vi "GateCrossing.vi"() -> ()   [LabVIEW 2024]
uses:
  class/mqtt/mqttTypedef/mqttSubscribeCluster.ctl
  class/mqtt/mqttTypedef/mqttQOSlevel.ctl
  class/mqtt/mqttTypedef/mqttBroker.ctl
  class/mqtt/mqttTypedef/mqttWillInformation.ctl
  class/mqtt/mqttTXqueue/mqttTXdataQueueFunction.ctl
  class/mqtt/mqttConfigFunction.ctl
  class/mqtt/mqttTXqueue/mqttRXsubscriptionEventFunction.ctl
  class/mqtt/mqttTypedef/mqttConnectionMeta.ctl
  <vilib>/Instr/_visa.llb/VISA Configure Serial Port (Instr).vi
  class/mqtt/mqtt.lvclass
panel:
  in  "stop":bool
  out "quit":bool
  in  "?":enum32{"HMI", "MQTT"}(tab)=enum."MQTT"
  out "Received String":string
  in  "Move Gate Down?":bool
  out "Sent Command":string
  out "?":bool
  in  "Send Command":bool
  in  "Toggle Buzzer?":bool
  in  "Toggle Lights?":bool
  in  "Enable HMI":bool
  out "valueSent 2":string
  in  "topic 2":string="/v1.6/devices/arduino/VAR_NAME"
  out "publishSuccess 2":bool
  in  "publish 2":bool
  out "value 2":string="0"
  out "autoPublish 2":bool
  out "valueSent":string
  in  "Enable Auto Publish":bool
  in  "subscribe":bool
  in  "topic":string="/v1.6/devices/arduino/VAR_NAME"
  out "publishSuccess":bool
  out "subscribeSuccess":bool
  in  "subscriptionInfo":T1[](array[typedef])=[{"Topic"="/v1.6/devices/arduino/VAR_NAME/lv", "QoS"=enum."At least once"}]
  in  "connect":bool
  in  "disconnect":bool
  out "RX Topic":string
  out "RX Value":string
  in  "publish":bool
  out "value":string="0"
  out "autoPublish":bool
  in  "broker":T3={"address"="industrial.api.ubidots.com", "port"=1883, "connTimeout"=30000, "writeTimeout"=2000, "readTimeout"=2000, "subTimeout"=300000}
  in  "client":string="SMRTTECH3CC3-STUDENT_NAME"
  in  "User Info":T4
  out "obstructrion":string
  out "gate_status":string
  in  "Enable Auto Publish 2":bool
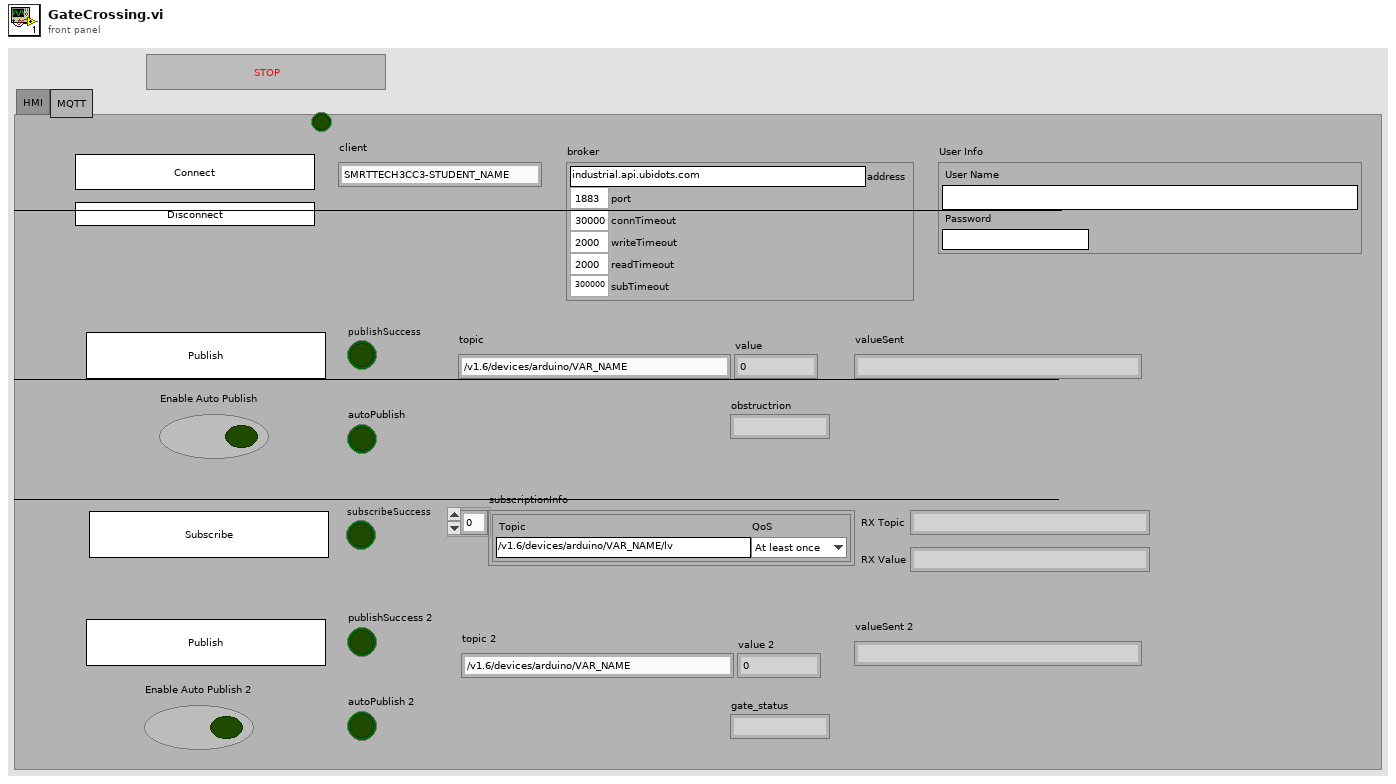
[diagram p1: front panel]
types:
  T1 = typedef "mqttSubscribeCluster.ctl" = cluster{"Topic":string, "QoS":T2}
  T2 = typedef "mqttQOSlevel.ctl" = enum8{"At most once", "At least once", "Exactly once", "Reserved"}
  T3 = typedef "mqttBroker.ctl" = cluster{"address":string, "port":u16, "connTimeout":i32, "writeTimeout":i32, "readTimeout":i32, "subTimeout":i32}
  T4 = typedef "mqttWillInformation.ctl" = cluster{"User Name":string, "Password":string}
  T5 = typedef "mqttRXsubscriptionEventFunction.ctl" = enum16{"init", "deinit", "getEventRef", "event"}
  T6 = typedef "mqtt.lvclass/mqttConfigFunction.ctl" = enum16{"init", "deinit", "set", "get"}
  T7 = typedef "mqttTXdataQueueFunction.ctl" = enum16{"init", "deinit", "getQueue", "enqueue"}
  T8 = enum8{"Enabled", "Disabled", "Disabled and Grayed Out"}
  T9 = typedef "mqttConnectionMeta.ctl" = cluster{"retain":bool, "duplicate":bool, "qos":T2}
  T10 = typedef "mqttConnectionStatus.ctl" = enum16{"Connection accepted", "Connection refused: unacceptable protocol version", "Connection refused: identifier rejected", "Connection refused: Server unavailable", "Connection refused: bad user name or password", "Connection refused: not authorized"}
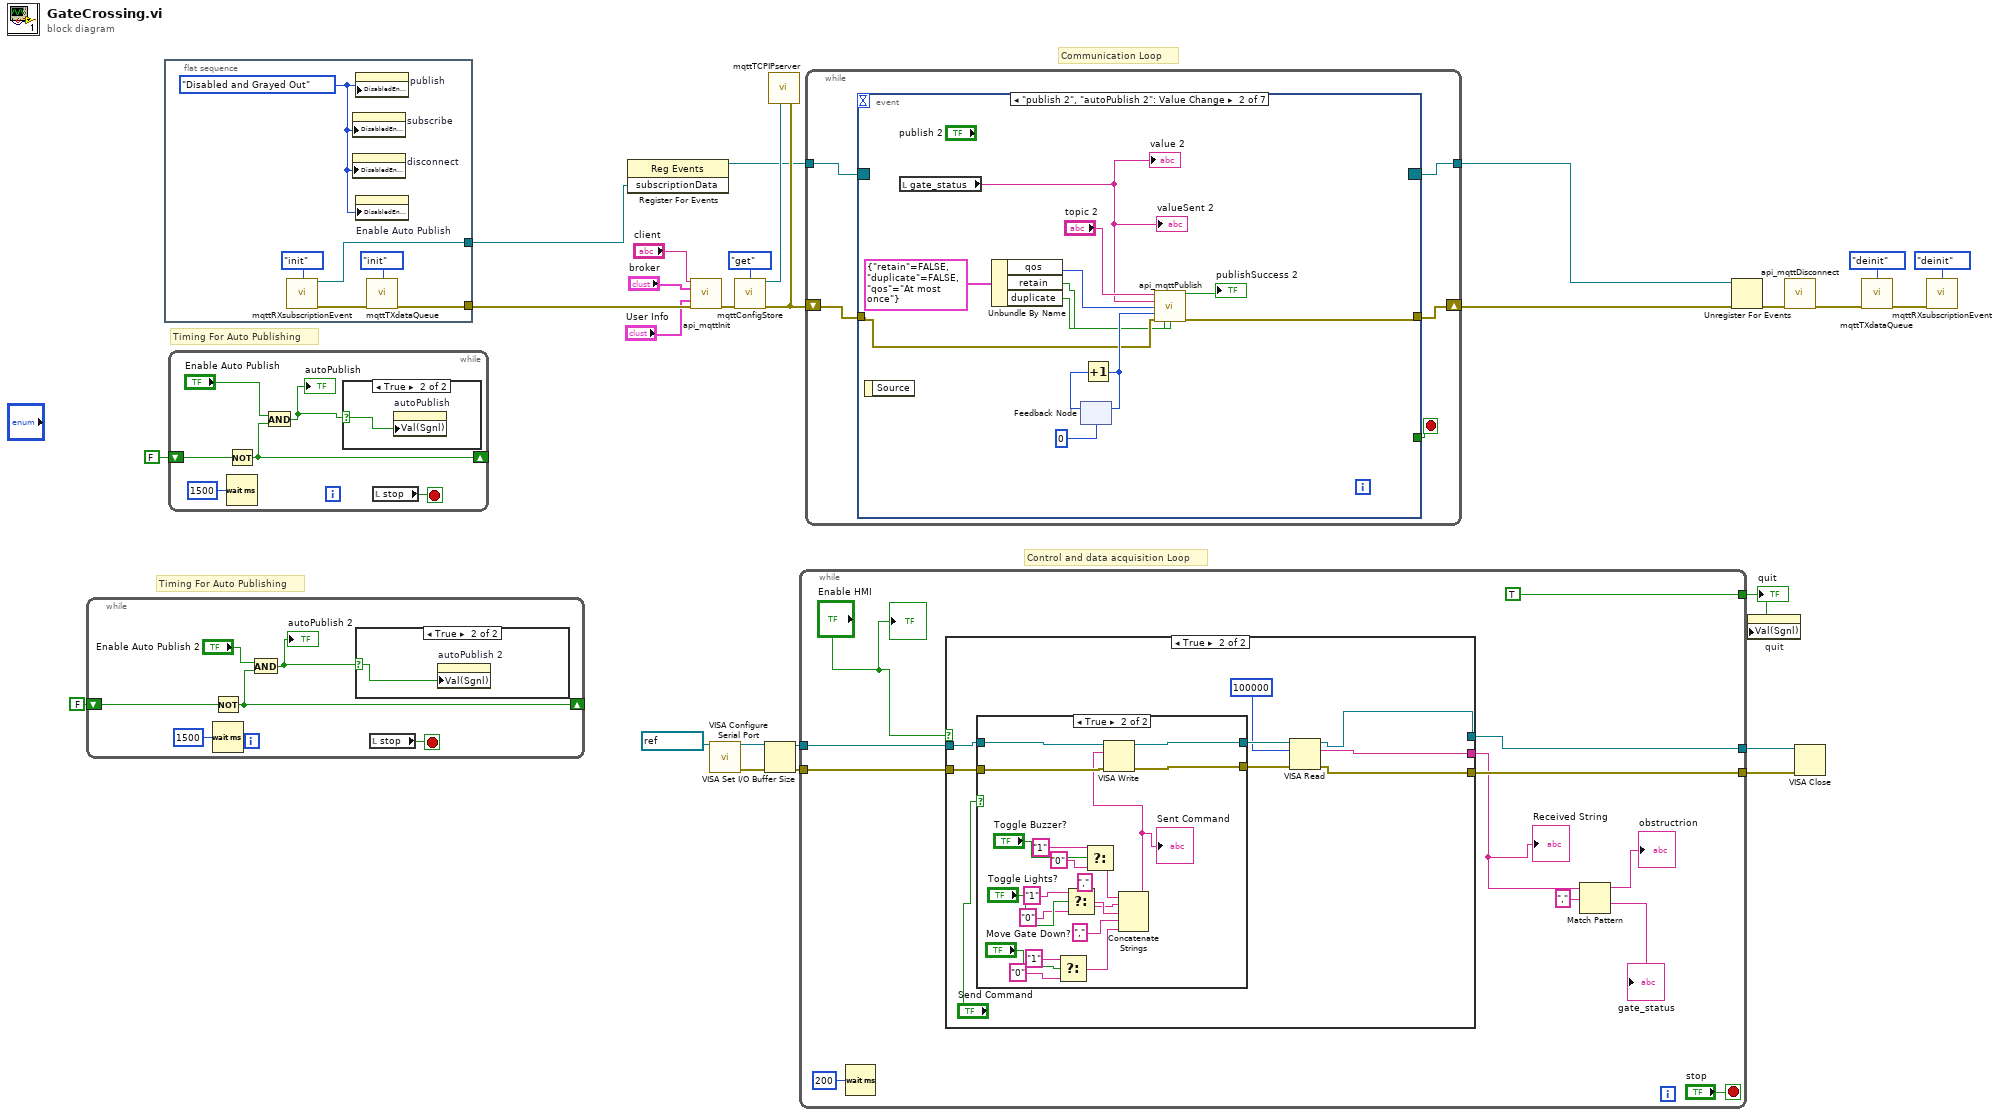
[diagram p0: block diagram]
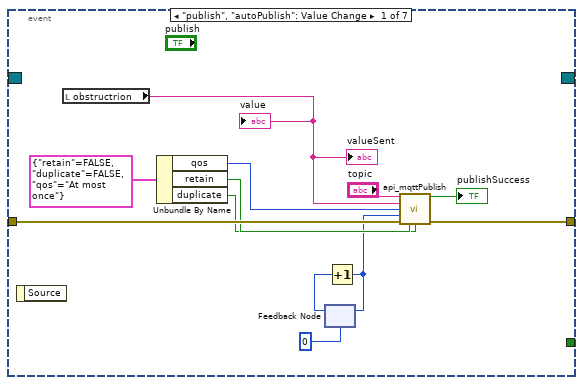
[diagram p6: hidden frame]
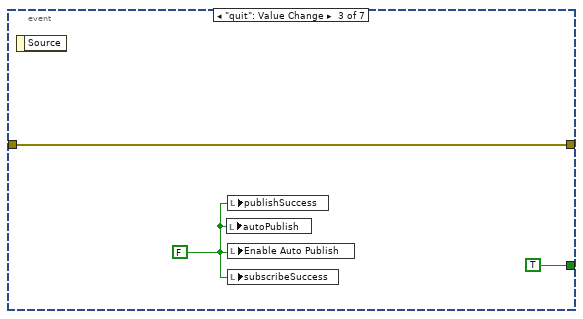
[diagram p7: hidden frame]
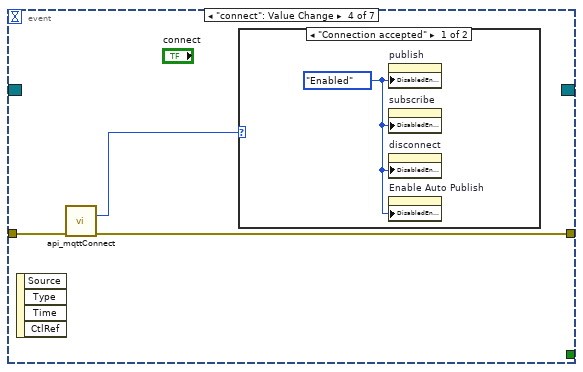
[diagram p8: hidden frame]
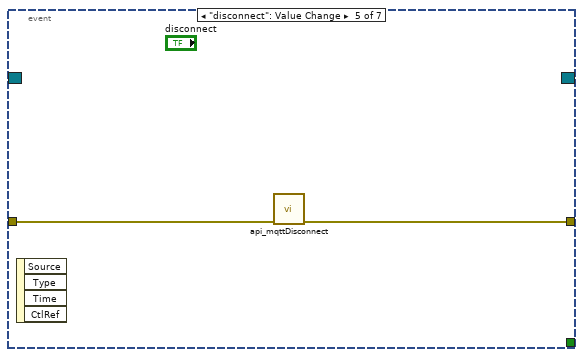
[diagram p10: hidden frame]
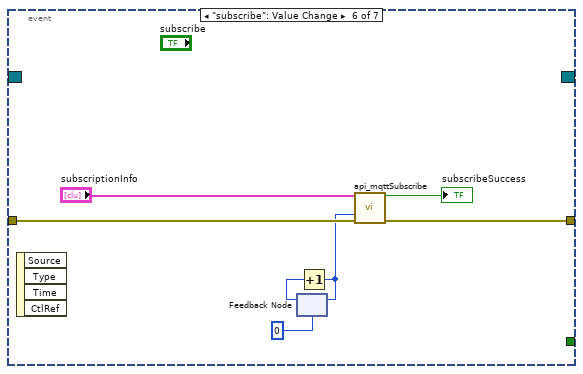
[diagram p11: hidden frame]
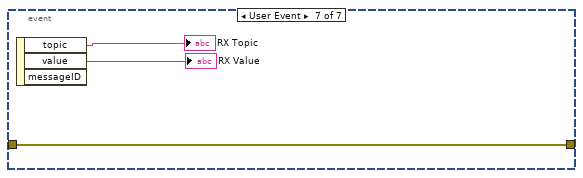
[diagram p12: hidden frame]
diagram:
  # "Timing For Auto Publishing"
  # "Timing For Auto Publishing"
  # "Control and data acquisition Loop"
  # "Communication Loop"
  n1 = while {
    shift-right: [w30] -> _
    shift-left: FALSE -> [w31]
    stop <- w32 stop-if-true
    n2 = Not(x=w31) -> (.not. x?=w30:bool)
    n3 = Wait (ms)(milliseconds to wait=u32 1500) -> ()  [unwired: 1 out]
    n4 = And(x="Enable Auto Publish 2", y=w30) -> (x .and. y?=w29:bool)
    "autoPublish 2" <- w29
    n5 = case shown="True" w29 {
      selector: w29 -> [_ w34]
      frame False {
      }
      frame True {
        n6 = property on="autoPublish 2" class="Bool"("Val(Sgnl)"=w34) -> ()  [unwired: 2 in, 2 out]
      }
    }
    n7 = local read "stop"() -> (w32:bool)
  }
  n8 = flat-sequence {
    tunnel: [w39] -> w26
    tunnel: [w36] -> w20
    frame #0 {
      w35 = T8."Disabled and Grayed Out" ("Disabled")
      n9 = call "mqttRXsubscriptionEvent.vi"("function"=mqttRXsubscriptionEventFunction."init") -> ("subscriptionData"=w36:refnum<user-event>, "error out"=w38:errorcluster)  [unwired: 13 in]
      n10 = property on="subscribe" class="Bool"("DisabledEnum"=w35) -> ()  [unwired: 2 in, 2 out]
      n11 = property on="disconnect" class="Bool"("DisabledEnum"=w35) -> ()  [unwired: 2 in, 2 out]
      n12 = property on="publish" class="Bool"("DisabledEnum"=w35) -> ()  [unwired: 2 in, 2 out]
      n13 = property on="Enable Auto Publish" class="Bool (strict)"("DisabledEnum"=w35) -> ()  [unwired: 2 in, 2 out]
      n14 = call "mqttTXdataQueue.vi"("function"=mqttTXdataQueueFunction."init", "error in (no error)"=w38) -> ("error out"=w39:errorcluster)  [unwired: 12 in, 1 out]
    }
  }
  n15 = while {
    shift-right: [w42] -> _
    shift-left: FALSE -> [w43]
    stop <- w44 stop-if-true
    n16 = Not(x=w43) -> (.not. x?=w42:bool)
    n17 = Wait (ms)(milliseconds to wait=u32 1500) -> ()  [unwired: 1 out]
    n18 = And(x="Enable Auto Publish", y=w42) -> (x .and. y?=w41:bool)
    "autoPublish" <- w41
    n19 = case shown="True" w41 {
      selector: w41 -> [_ w47]
      frame False {
      }
      frame True {
        n20 = property on="autoPublish" class="Bool"("Val(Sgnl)"=w47) -> ()  [unwired: 2 in, 2 out]
      }
    }
    n21 = local read "stop"() -> (w44:bool)
  }
  n22 = register-events(w20) -> (reference out=w19:refnum<event-registration>)  [unwired: 2 in, 1 out]
  n23 = call "api_mqttInit.vi"("client"="client", "broker"="broker", "User Info"="User Info", "error in (no error)"=w26) -> ("error out"=w24:errorcluster)  [unwired: 11 in]
  n24 = call-poly "VISA Configure Serial Port"("VISA resource name"=refnum<visa-resource-name> "COM5") -> ("VISA resource name out"=w7:refnum<visa-resource-name>, "error out"=w4:errorcluster)  [unwired: 13 in]
  n25 = call "mqttConfigStore.vi"("function"=mqttConfigFunction."get", "error in (no error)"=w24) -> ("mqtt.lvclass out"=w23:refnum<class "mqtt.lvclass">, "error out"=w22:errorcluster)  [unwired: 12 in]
  n26 = VISA Set I/O Buffer Size(VISA resource name=w7, error in (no error)=w4) -> (VISA resource name out=w6:refnum<visa-resource-name>, error out=w3:errorcluster)  [unwired: 2 in]
  n27 = call "mqttTCPIPserver.vi"("mqtt.lvclass"=w23, "error in (no error)"=w22) -> ()  [unwired: 12 in, 2 out]
  n28 = while {
    tunnel: [TRUE] -> w9
    tunnel: w6 -> [w56]
    tunnel: [w52] -> w5
    tunnel: w3 -> [w55]
    tunnel: [w54] -> w2
    stop <- "stop" stop-if-true
    n29 = Wait (ms)(milliseconds to wait=u32 200) -> ()  [unwired: 1 out]
    n30 = case shown="True" "Enable HMI" {
      tunnel: w56 -> [w61 w65]
      tunnel: w55 -> [w60 w66]
      tunnel: [w60 w70] -> w54
      tunnel: [w61 w69] -> w52
      tunnel: [_ w68] -> w48
      frame False {
      }
      frame True {
        n31 = case shown="True" "Send Command" {
          tunnel: [w71 w91] -> w67
          tunnel: w66 -> [w71 w90]
          tunnel: [w72 w89] -> w63
          tunnel: w65 -> [w72 w88]
          frame False {
          }
          frame True {
            n32 = Select(t="1", s="Move Gate Down?", f="0") -> (s? t:f=w76:string)
            n33 = Select(t="1", s="Toggle Lights?", f="0") -> (s? t:f=w77:string)
            n34 = Select(t="1", s="Toggle Buzzer?", f="0") -> (s? t:f=w78:string)
            n35 = Concatenate Strings(w78, ",", w77, ",", w76) -> (w79:string)
            "Sent Command" <- w79
            n36 = VISA Write(VISA resource name=w88, write buffer=w79, error in (no error)=w90) -> (VISA resource name out=w89:refnum<visa-resource-name>, error out=w91:errorcluster)  [unwired: 1 out]
          }
        }
        n37 = VISA Read(VISA resource name=w63, byte count=u32 100000, error in (no error)=w67) -> (VISA resource name out=w69:refnum<visa-resource-name>, read buffer=w68:string, error out=w70:errorcluster)  [unwired: 1 out]
      }
    }
    "Received String" <- w48
    n38 = Match Pattern(string=w48, regular expression=",") -> (before substring=→"obstructrion":string, after substring=→"gate_status":string)  [unwired: 1 in, 2 out]
    "?" <- "Enable HMI"
  }
  "quit" <- w9
  n39 = while {
    shift-right: [w96] -> w16
    shift-left: w22 -> [w95]
    tunnel: w19 -> [w93]
    tunnel: [w92] -> w14
    stop <- w94 stop-if-true
    n40 = event shown="[1] \"publish 2\", \"autoPublish 2\": Value Change" {
      selector: w93 -> [_ _ _ _ _ _ _]
      dyn-events: [_ _ _ _ _ _ _] -> w92
      timeout: _ -> [_ _ _ _ _ _ _]
      tunnel: [w107 w115 w122 w125 w128 w134 w139] -> w96
      tunnel: w95 -> [w108 w116 w122 w126 w129 w133 w139]
      tunnel: [_ _ TRUE _ _ _ _] -> w94
      event "publish", "autoPublish": Value Change {
        n41 = event-data() -> ()  [unwired: 1 in, 1 out]
        n42 = local read "obstructrion"() -> (w97:string)
        "value" <- w97
        "valueSent" <- w97
        n43 = Unbundle By Name(T9 {"retain"=FALSE, "duplicate"=FALSE, "qos"=enum."At most once"} ("connMeta")) -> ("qos"=w103:T2, "retain"=w102:bool, "duplicate"=w101:bool)
        n44 = feedback #1(u16 0) -> (w99:u16)
        n45 = Increment(x=w99) -> (x+1=w98:u16)
        n46 = feedback-in #1(w98) -> ()
        n47 = call "api_mqttPublish.vi"("topic"="topic", "value"=w97, "QoS (At most once)"=w103, "messageID"=w98, "error in (no error)"=w108, "retain(F)"=w102, "duplicate(F)"=w101) -> ("success"=→"publishSuccess":bool, "error out"=w107:errorcluster)  [unwired: 7 in]
      }
      event "publish 2", "autoPublish 2": Value Change {
        n48 = event-data() -> ()  [unwired: 1 in, 1 out]
        n49 = local read "gate_status"() -> (w109:string)
        "value 2" <- w109
        "valueSent 2" <- w109
        n50 = Unbundle By Name(T9 {"retain"=FALSE, "duplicate"=FALSE, "qos"=enum."At most once"} ("connMeta")) -> ("qos"=w114:T2, "retain"=w112:bool, "duplicate"=w113:bool)
        n51 = feedback #2(u16 0) -> (w118:u16)
        n52 = Increment(x=w118) -> (x+1=w117:u16)
        n53 = feedback-in #2(w117) -> ()
        n54 = call "api_mqttPublish.vi"("topic"="topic 2", "value"=w109, "QoS (At most once)"=w114, "messageID"=w117, "error in (no error)"=w116, "retain(F)"=w112, "duplicate(F)"=w113) -> ("success"=→"publishSuccess 2":bool, "error out"=w115:errorcluster)  [unwired: 7 in]
      }
      event "quit": Value Change {
        w121 = FALSE ("Enable Auto Publish")
        n55 = event-data() -> ()  [unwired: 1 in, 1 out]
        n56 = local write "autoPublish"(w121) -> ()
        n57 = local write "publishSuccess"(w121) -> ()
        n58 = local write "Enable Auto Publish"(w121) -> ()
        n59 = local write "subscribeSuccess"(w121) -> ()
      }
      event "connect": Value Change {
        n60 = event-data() -> ()  [unwired: 1 in, 4 out]
        n61 = call "api_mqttConnect.vi"("error in (no error)"=w126) -> ("connStatus"=w124:T10, "error out"=w125:errorcluster)  [unwired: 11 in, 2 out]
        n62 = case shown="\"Connection accepted\"" w124 {
          frame "Connection accepted" {
            w127 = T8."Enabled" ("Disabled")
            n63 = property on="publish" class="Bool"("DisabledEnum"=w127) -> ()  [unwired: 2 in, 2 out]
            n64 = property on="subscribe" class="Bool"("DisabledEnum"=w127) -> ()  [unwired: 2 in, 2 out]
            n65 = property on="disconnect" class="Bool"("DisabledEnum"=w127) -> ()  [unwired: 2 in, 2 out]
            n66 = property on="Enable Auto Publish" class="Bool (strict)"("DisabledEnum"=w127) -> ()  [unwired: 2 in, 2 out]
          }
          frame Default {
          }
        }
      }
      event "disconnect": Value Change {
        n67 = event-data() -> ()  [unwired: 1 in, 4 out]
        n68 = call "api_mqttDisconnect.vi"("error in (no error)"=w129) -> ("error out"=w128:errorcluster)  [unwired: 13 in, 1 out]
      }
      event "subscribe": Value Change {
        n69 = event-data() -> ()  [unwired: 1 in, 4 out]
        n70 = feedback #3(u16 0) -> (w131:u16)
        n71 = Increment(x=w131) -> (x+1=w130:u16)
        n72 = feedback-in #3(w130) -> ()
        n73 = call "api_mqttSubscribe.vi"("subscriptionInfo"="subscriptionInfo", "messageID"=w130, "error in (no error)"=w133) -> ("success"=→"subscribeSuccess":bool, "error out"=w134:errorcluster)  [unwired: 11 in]
      }
      event User Event {
        n74 = event-data() -> ("topic"=→"RX Topic":string, "value"=→"RX Value":string)  [unwired: 1 in, 1 out]
      }
    }
  }
  n75 = Unregister For Events(event registration refnum=w14, error in=w16) -> (error out=w15:errorcluster)
  n76 = property on="quit" class="Bool"("Val(Sgnl)"=w9) -> ()  [unwired: 2 in, 2 out]
  n77 = call "api_mqttDisconnect.vi"("error in (no error)"=w15) -> ("error out"=w21:errorcluster)  [unwired: 13 in, 1 out]
  n78 = VISA Close(VISA resource name=w5, error in (no error)=w2) -> ()  [unwired: 1 out]
  n79 = call "mqttTXdataQueue.vi"("function"=mqttTXdataQueueFunction."deinit", "error in (no error)"=w21) -> ("error out"=w17:errorcluster)  [unwired: 12 in, 1 out]
  n80 = call "mqttRXsubscriptionEvent.vi"("function"=mqttRXsubscriptionEventFunction."deinit", "error in (no error)"=w17) -> ()  [unwired: 12 in, 2 out]
